vi "FlatToRichlv_python_grpc_webui_demo_v1_UpdateSetPointRequest.vi"(5 "OutputClusterType":T1, 11 "InputCluster":T2) -> (3 "OutputCluster":T1)   [LabVIEW 2020, in "thermal-chamber-controller_server.lvlib"]
uses:
  thermal-chamber-controller_server.lvlib
  lv_python_grpc_webui_demo_v1_UpdateSetPointRequest_Flat.ctl
  lv_python_grpc_webui_demo_v1_UpdateSetPointRequest.ctl
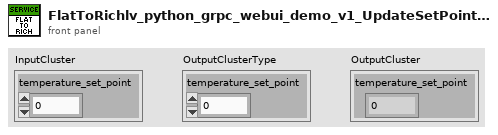
[diagram p1: front panel]
types:
  T1 = typedef "thermal-chamber-controller_server.lvlib/lv_python_grpc_webui_demo_v1_UpdateSetPointRequest.ctl" = cluster{"temperature_set_point":dbl}
  T2 = typedef "thermal-chamber-controller_server.lvlib/lv_python_grpc_webui_demo_v1_UpdateSetPointRequest_Flat.ctl" = cluster{"temperature_set_point":dbl}
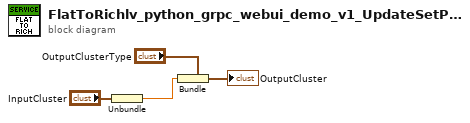
[diagram p0: block diagram]
diagram:
  n1 = Unbundle "Unbundle"("InputCluster") -> ("temperature_set_point"=w1:dbl)
  n2 = Bundle "Bundle"(cluster="OutputClusterType", "temperature_set_point"=w1) -> (→"OutputCluster":T1)
